vi "Create Message Data Clusters (simple).vi"(8 "error in (no error)":errorcluster, 9 "generate serialization helpers":bool, 10 "message metadata":T1, 11 "library in":refnum<vi>) -> (0 "error out":errorcluster, 3 "library out":refnum<vi>)   [LabVIEW 2019, in "gRPC Template Creation Utility.lvlib"]
uses:
  gRPC Template Creation Utility.lvlib
  TypeDefs/Message Metadata (Scripting).ctl
  TypeDefs/Message Element Metadata (Scripting).ctl
  TypeDefs/Message Element Type.ctl
  Oneof API/OneOf Constants/OneOfConstantsEnum.ctl
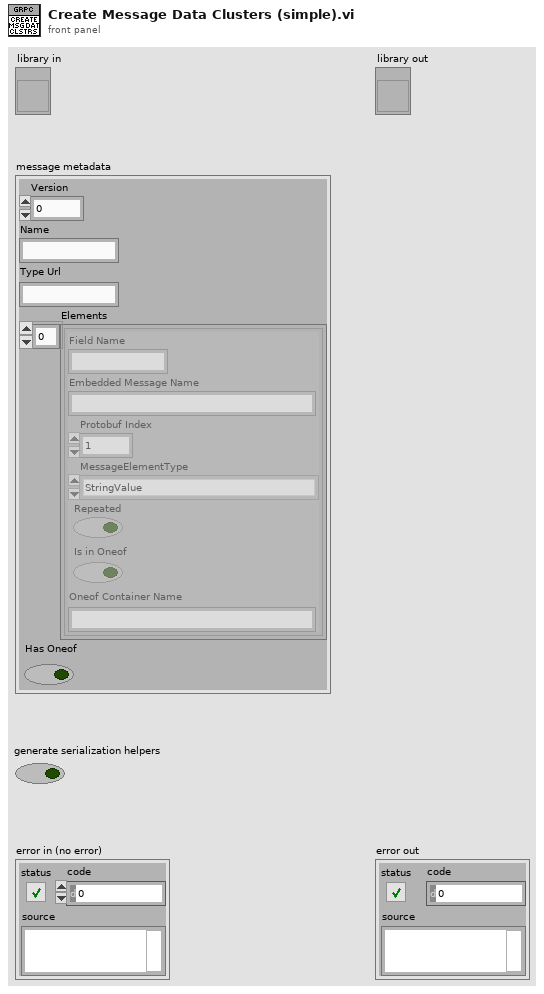
[diagram p1: front panel]
types:
  T1 = typedef "gRPC Template Creation Utility.lvlib/Message Metadata (Scripting).ctl" = cluster{"Version":i32, "Name":string, "Type Url":string, "Elements":T2[], "Has Oneof":bool}
  T2 = typedef "gRPC Template Creation Utility.lvlib/Message Element Metadata (Scripting).ctl" = cluster{"Field Name":string, "Embedded Message Name":string, "Protobuf Index":i32, "MessageElementType":T3, "Repeated":bool, "Is in Oneof":bool, "Oneof Container Name":string}
  T3 = typedef "gRPC Template Creation Utility.lvlib/Message Element Type.ctl" = enum32{"Int32Value", "FloatValue", "DoubleValue", "BoolValue", "StringValue", "MessageValue", "Int64Value", "UInt32Value", "UInt64Value", "EnumValue", "Bytes", "Fixed64", "Fixed32", "SFixed64", "SFixed32", "SInt64", "SInt32"}
  T4 = typedef "gRPC Template Creation Utility.lvlib/OneOfConstantsEnum.ctl" = enum16{"FlatToRichVIPrefix", "RichToFlatVIPrefix", "FlatTypeDefSuffix"}
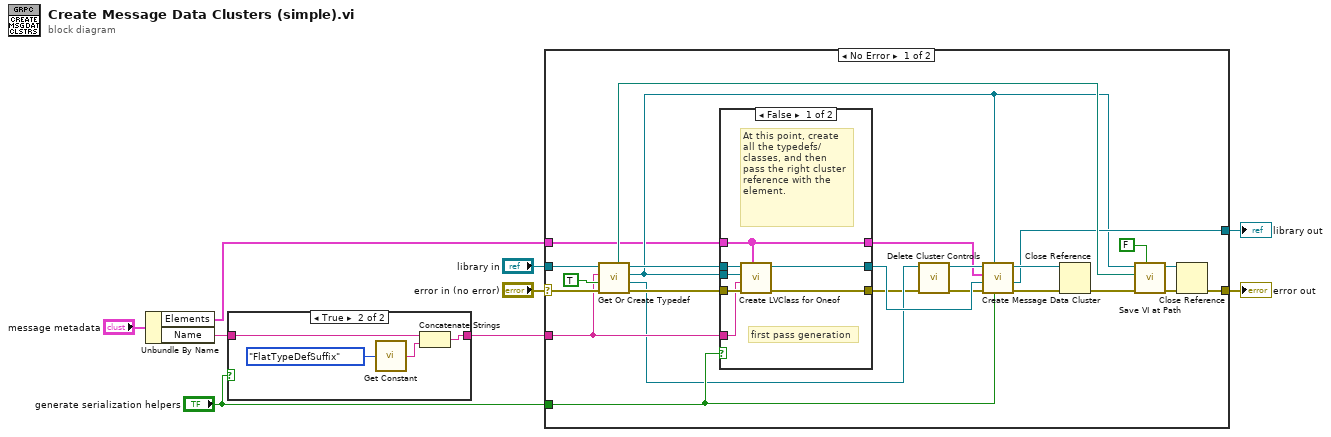
[diagram p0: block diagram]
diagram:
  n1 = Unbundle By Name("message metadata") -> ("Elements"=w4:T2[], "Name"=w1:string)
  n2 = case shown="True" "generate serialization helpers" {
    tunnel: w1 -> [w10 w14]
    tunnel: [w10 w13] -> w3
    frame False {
    }
    frame True {
      n3 = call "Get Constant.vi"("Selection"=OneOfConstantsEnum."FlatTypeDefSuffix") -> ("String"=w11:string)
      n4 = Concatenate Strings(w14, w11) -> (w13:string)
    }
  }
  n5 = case shown="No Error" "error in (no error)" {
    selector: "error in (no error)" -> [w35 w49]
    tunnel: "library in" -> [w38 w50]
    tunnel: [w30 w49] -> w8
    tunnel: [w24 w50] -> w7
    tunnel: w3 -> [w22 _]
    tunnel: w4 -> [w21 _]
    tunnel: "generate serialization helpers" -> [w20 _]
    frame No Error {
      n6 = call "Get Or Create Typedef.vi"("error in (no error)"=w35, "Create cluster inside Typedef?"=TRUE, "Name"=w22, "Library in"=w38) -> ("error out"=w26:errorcluster, "Cluster ref out"=w19:refnum<vi>, "VI ref out"=w23:refnum<vi>, "Library out"=w27:refnum<vi>, "Path"=w29:path)  [unwired: 3 in]
      n7 = case shown="False" w20 {
        tunnel: w27 -> [w45 w48]
        tunnel: w26 -> [w44 w47]
        tunnel: [w43 w47] -> w18
        tunnel: [w42 w48] -> w25
        tunnel: w23 -> [w41 _]
        tunnel: w22 -> [w40 _]
        tunnel: w21 -> [w39 w46]
        tunnel: [w39 w46] -> w15
        frame False {
          # "first pass generation"
          # "At this point, create all the typedefs/classes, and then\npass the right cluster reference with the element."
          n8 = call "Create LVClass for Oneof.vi"("Message Elements"=w39, "error in (no error)"=w44, "Message Name"=w40, "Parent Message Typedef"=w41, "Library"=w45) -> ("error out"=w43:errorcluster, "Library"=w42:refnum<vi>)  [unwired: 5 in]
        }
        frame True {
        }
      }
      n9 = call "Delete Cluster Controls.vi"("error in (no error)"=w18, "Cluster in"=w19) -> ("error out"=w17:errorcluster, "Cluster out"=w16:refnum<vi>)  [unwired: 8 in]
      n10 = call "Create Message Data Cluster.vi"("generate converters"=w20, "owning typedef"=w23, "error in (no error)"=w17, "library in"=w25, "message element metafata"=w15, "cluster in"=w16) -> ("error out"=w34:errorcluster, "library out"=w24:refnum<vi>, "cluster out"=w32:refnum<vi>)  [unwired: 3 in]
      n11 = Close Reference(reference=w32, error in (no error)=w34) -> (error out=w33:errorcluster)
      n12 = call "Save VI at Path.vi"("Override Existing? (T)"=FALSE, "error in (no error)"=w33, "Path"=w29, "VI in"=w23) -> ("error out"=w37:errorcluster, "VI out"=w36:refnum<vi>)  [unwired: 5 in, 1 out]
      n13 = Close Reference(reference=w36, error in (no error)=w37) -> (error out=w30:errorcluster)
    }
    frame Error {
    }
  }
  "error out" <- w8
  "library out" <- w7
